vi "[ce] INI - RW Control Values.vi"(6 "cmd (load)":enum16{"load", "save"}(ring), 7 "Section":string="GENERAL", 8 "error in":errorcluster, 10 "Ctrl refnums":refnum<vi>[](array[refnum]), 11 "INI refnum":T1) -> (0 "error out":errorcluster, 3 "dup INI refnum":T1)   [LabVIEW 2021]
doc: "::: CalcExpress Toolkit :::\nCopyright (c) 2000-2026 Konstantin Shifershteyn. All rights reserved."
uses:
  <vilib>/Utility/config.llb/Config Data RefNum.ctl
  <vilib>/Utility/config.llb/Write Key (Path).vi
  <vilib>/Utility/config.llb/Write Key (String).vi
  <vilib>/Utility/config.llb/Write Key (Boolean).vi
  <vilib>/Utility/config.llb/Write Key (U32).vi
  <vilib>/Utility/config.llb/Write Key (I32).vi
  <vilib>/Utility/config.llb/Write Key (Double).vi
  <vilib>/Utility/config.llb/Read Key (Path).vi
  <vilib>/Utility/config.llb/Read Key (String).vi
  <vilib>/Utility/config.llb/Read Key (Boolean).vi
  <vilib>/Utility/config.llb/Read Key (U32).vi
  <vilib>/Utility/config.llb/Read Key (I32).vi
  <vilib>/Utility/config.llb/Read Key (Double).vi
  <vilib>/Utility/config.llb/NI_LVConfig.lvlib
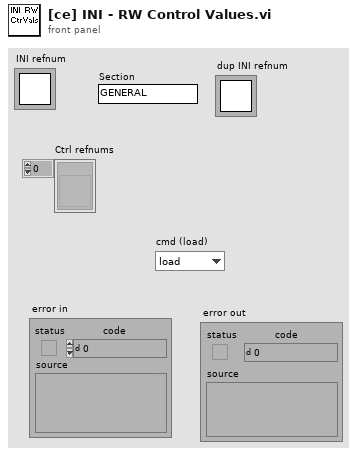
[diagram p1: front panel]
types:
  T1 = typedef "NI_LVConfig.lvlib/Config Data RefNum.ctl" = refnum<k1>
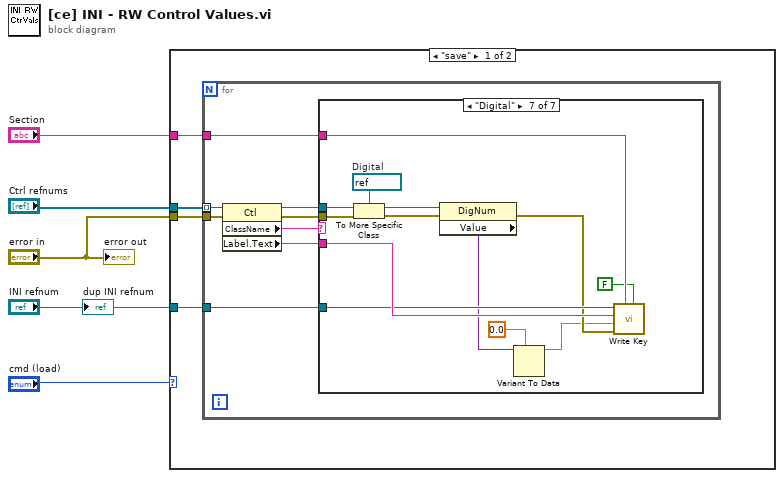
[diagram p0: block diagram]
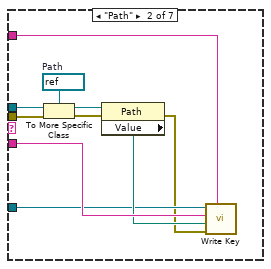
[diagram p3: hidden frame]
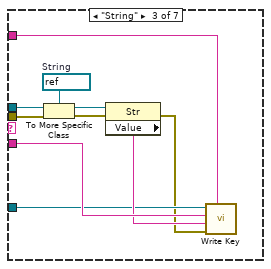
[diagram p4: hidden frame]
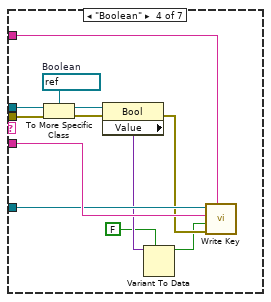
[diagram p5: hidden frame]
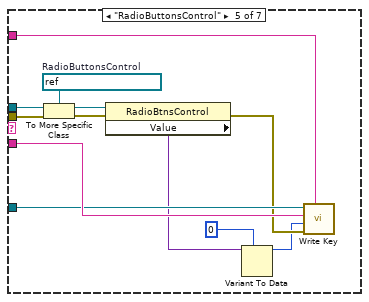
[diagram p6: hidden frame]
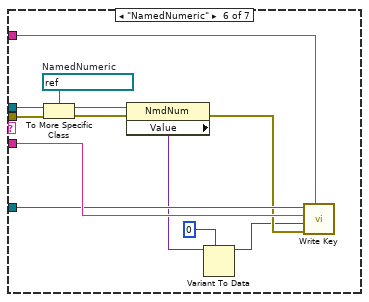
[diagram p7: hidden frame]
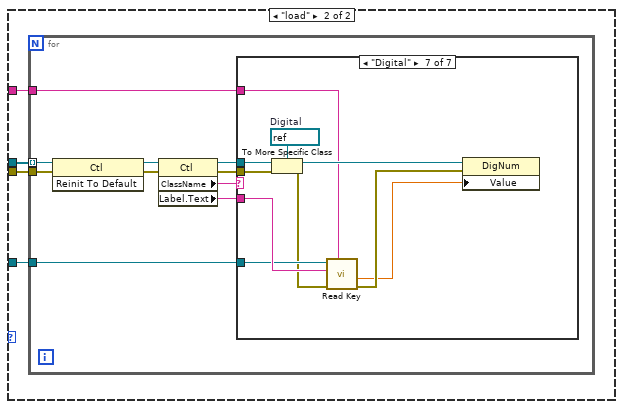
[diagram p8: hidden frame]
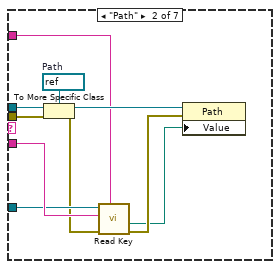
[diagram p10: hidden frame]
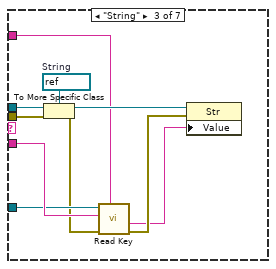
[diagram p11: hidden frame]
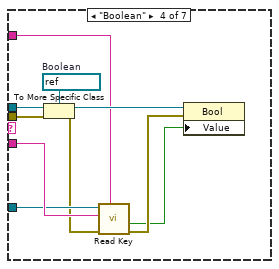
[diagram p12: hidden frame]
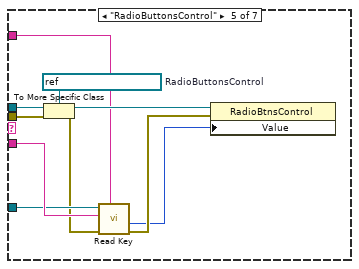
[diagram p13: hidden frame]
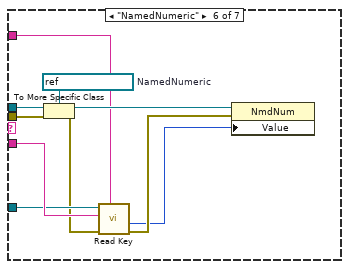
[diagram p14: hidden frame]
diagram:
  n1 = case shown="\"save\"" "cmd (load)" {
    tunnel: "Ctrl refnums" -> [w9 w92]
    tunnel: "error in" -> [w8 w91]
    tunnel: "INI refnum" -> [w7 w90]
    tunnel: "Section" -> [w6 w89]
    frame "save" {
      n2 = for {
        tunnel: w9 -> [w14] mode=indexing
        tunnel: w7 -> [w13]
        tunnel: w8 -> [w11]
        tunnel: w6 -> [w10]
        n3 = property class="Ctl"(reference=w14, error in=w11) -> (reference out=w16:refnum<vi>, error out=w12:errorcluster, "ClassName"=w17:string, "Label.Text"=w15:string)
        n4 = case shown="\"Digital\"" w17 {
          selector: w17 -> [w19 _ _ _ _ _ _]
          tunnel: w16 -> [_ w29 w39 w51 w63 w75 w88]
          tunnel: w15 -> [w18 w26 w36 w48 w60 w72 w85]
          tunnel: w13 -> [_ w24 w34 w47 w59 w71 w84]
          tunnel: w12 -> [_ w23 w33 w46 w58 w70 w83]
          tunnel: w10 -> [_ w20 w30 w43 w55 w67 w80]
          frame Default {
            n5 = flat-sequence {
              tunnel: w19 -> [_]
              tunnel: w18 -> [_]
              frame #0 {
              }
            }
          }
          frame "Path" {
            w27 = refnum<vi> refnum  # Path
            n6 = To More Specific Class(target class=w27, reference=w29, error in=w23) -> (specific class reference=w28:refnum<vi>, error out=w22:errorcluster)
            n7 = property class="Path"(reference=w28, error in=w22) -> (error out=w21:errorcluster, "Value"=w25:path)  [unwired: 1 out]
            n8 = call-poly <vilib>:"Write Key.vi"("section"=w20, "error in (no error)"=w21, "value"=w25, "key"=w26, "refnum"=w24) -> ()  [unwired: 4 in, 3 out]
          }
          frame "String" {
            w37 = refnum<vi> refnum  # String
            n9 = To More Specific Class(target class=w37, reference=w39, error in=w33) -> (specific class reference=w38:refnum<vi>, error out=w32:errorcluster)
            n10 = property class="Str"(reference=w38, error in=w32) -> (error out=w31:errorcluster, "Value"=w35:string)  [unwired: 1 out]
            n11 = call-poly <vilib>:"Write Key.vi"("section"=w30, "error in (no error)"=w31, "value"=w35, "key"=w36, "refnum"=w34) -> ()  [unwired: 4 in, 3 out]
          }
          frame "Boolean" {
            w49 = refnum<vi> refnum  # Boolean
            n12 = To More Specific Class(target class=w49, reference=w51, error in=w46) -> (specific class reference=w50:refnum<vi>, error out=w45:errorcluster)
            n13 = property class="Bool"(reference=w50, error in=w45) -> (error out=w44:errorcluster, "Value"=w42:variant)  [unwired: 1 out]
            n14 = Variant To Data(type=FALSE, Variant=w42) -> (data=w40:bool)  [unwired: 1 in, 1 out]
            n15 = call-poly <vilib>:"Write Key.vi"("section"=w43, "error in (no error)"=w44, "value"=w40, "key"=w48, "refnum"=w47) -> ()  [unwired: 4 in, 3 out]
          }
          frame "RadioButtonsControl" {
            w61 = refnum<vi> refnum  # RadioButtonsControl
            n16 = To More Specific Class(target class=w61, reference=w63, error in=w58) -> (specific class reference=w62:refnum<vi>, error out=w57:errorcluster)
            n17 = property class="RadioBtnsControl"(reference=w62, error in=w57) -> (error out=w56:errorcluster, "Value"=w54:variant)  [unwired: 1 out]
            n18 = Variant To Data(type=u32 0, Variant=w54) -> (data=w52:u32)  [unwired: 1 in, 1 out]
            n19 = call-poly <vilib>:"Write Key.vi"("section"=w55, "error in (no error)"=w56, "value"=w52, "key"=w60, "refnum"=w59) -> ()  [unwired: 4 in, 3 out]
          }
          frame "NamedNumeric" {
            w73 = refnum<vi> refnum  # NamedNumeric
            n20 = To More Specific Class(target class=w73, reference=w75, error in=w70) -> (specific class reference=w74:refnum<vi>, error out=w69:errorcluster)
            n21 = property class="NmdNum"(reference=w74, error in=w69) -> (error out=w68:errorcluster, "Value"=w66:variant)  [unwired: 1 out]
            n22 = Variant To Data(type=0, Variant=w66) -> (data=w64:i32)  [unwired: 1 in, 1 out]
            n23 = call-poly <vilib>:"Write Key.vi"("section"=w67, "error in (no error)"=w68, "value"=w64, "key"=w72, "refnum"=w71) -> ()  [unwired: 4 in, 3 out]
          }
          frame "Digital" {
            w86 = refnum<vi> refnum  # Digital
            n24 = To More Specific Class(target class=w86, reference=w88, error in=w83) -> (specific class reference=w87:refnum<vi>, error out=w82:errorcluster)
            n25 = property class="DigNum"(reference=w87, error in=w82) -> (error out=w81:errorcluster, "Value"=w79:variant)  [unwired: 1 out]
            n26 = Variant To Data(type=0.0, Variant=w79) -> (data=w77:dbl)  [unwired: 1 in, 1 out]
            n27 = call-poly <vilib>:"Write Key.vi"("use system decimal point (T)"=FALSE, "section"=w80, "error in (no error)"=w81, "value"=w77, "key"=w85, "refnum"=w84) -> ()  [unwired: 3 in, 3 out]
          }
        }
      }
    }
    frame "load" {
      n28 = for {
        tunnel: w92 -> [w96] mode=indexing
        tunnel: w90 -> [w99]
        tunnel: w91 -> [w94]
        tunnel: w89 -> [w97]
        n29 = invoke class="Ctl" method="Reinit To Default"(reference=w96, error in=w94) -> (reference out=w95:refnum<vi>, error out=w93:errorcluster)  [unwired: 1 in, 1 out]
        n30 = property class="Ctl"(reference=w95, error in=w93) -> (reference out=w101:refnum<vi>, error out=w98:errorcluster, "ClassName"=w102:string, "Label.Text"=w100:string)
        n31 = case shown="\"Digital\"" w102 {
          tunnel: w101 -> [_ w112 w122 w132 w142 w152 w162]
          tunnel: w100 -> [_ w109 w119 w129 w139 w149 w159]
          tunnel: w99 -> [_ w108 w118 w128 w138 w148 w158]
          tunnel: w98 -> [_ w107 w117 w127 w137 w147 w157]
          tunnel: w97 -> [_ w104 w114 w124 w134 w144 w154]
          frame Default {
          }
          frame "Path" {
            w110 = refnum<vi> refnum  # Path
            n32 = To More Specific Class(target class=w110, reference=w112, error in=w107) -> (specific class reference=w111:refnum<vi>, error out=w106:errorcluster)
            n33 = call-poly <vilib>:"Read Key.vi"("section"=w104, "error in (no error)"=w106, "key"=w109, "refnum"=w108) -> ("error out"=w105:errorcluster, "value"=w103:path)  [unwired: 4 in, 2 out]
            n34 = property class="Path"(reference=w111, error in=w105, "Value"=w103) -> ()  [unwired: 2 out]
          }
          frame "String" {
            w120 = refnum<vi> refnum  # String
            n35 = To More Specific Class(target class=w120, reference=w122, error in=w117) -> (specific class reference=w121:refnum<vi>, error out=w116:errorcluster)
            n36 = call-poly <vilib>:"Read Key.vi"("section"=w114, "error in (no error)"=w116, "key"=w119, "refnum"=w118) -> ("error out"=w115:errorcluster, "value"=w113:string)  [unwired: 4 in, 2 out]
            n37 = property class="Str"(reference=w121, error in=w115, "Value"=w113) -> ()  [unwired: 2 out]
          }
          frame "Boolean" {
            w130 = refnum<vi> refnum  # Boolean
            n38 = To More Specific Class(target class=w130, reference=w132, error in=w127) -> (specific class reference=w131:refnum<vi>, error out=w126:errorcluster)
            n39 = call-poly <vilib>:"Read Key.vi"("section"=w124, "error in (no error)"=w126, "key"=w129, "refnum"=w128) -> ("error out"=w125:errorcluster, "value"=w123:bool)  [unwired: 4 in, 2 out]
            n40 = property class="Bool"(reference=w131, error in=w125, "Value"=w123) -> ()  [unwired: 2 out]
          }
          frame "RadioButtonsControl" {
            w140 = refnum<vi> refnum  # RadioButtonsControl
            n41 = To More Specific Class(target class=w140, reference=w142, error in=w137) -> (specific class reference=w141:refnum<vi>, error out=w136:errorcluster)
            n42 = call-poly <vilib>:"Read Key.vi"("section"=w134, "error in (no error)"=w136, "key"=w139, "refnum"=w138) -> ("error out"=w135:errorcluster, "value"=w133:u32)  [unwired: 4 in, 2 out]
            n43 = property class="RadioBtnsControl"(reference=w141, error in=w135, "Value"=w133) -> ()  [unwired: 2 out]
          }
          frame "NamedNumeric" {
            w150 = refnum<vi> refnum  # NamedNumeric
            n44 = To More Specific Class(target class=w150, reference=w152, error in=w147) -> (specific class reference=w151:refnum<vi>, error out=w146:errorcluster)
            n45 = call-poly <vilib>:"Read Key.vi"("section"=w144, "error in (no error)"=w146, "key"=w149, "refnum"=w148) -> ("error out"=w145:errorcluster, "value"=w143:i32)  [unwired: 4 in, 2 out]
            n46 = property class="NmdNum"(reference=w151, error in=w145, "Value"=w143) -> ()  [unwired: 2 out]
          }
          frame "Digital" {
            w160 = refnum<vi> refnum  # Digital
            n47 = To More Specific Class(target class=w160, reference=w162, error in=w157) -> (specific class reference=w161:refnum<vi>, error out=w156:errorcluster)
            n48 = call-poly <vilib>:"Read Key.vi"("section"=w154, "error in (no error)"=w156, "key"=w159, "refnum"=w158) -> ("error out"=w155:errorcluster, "value"=w153:dbl)  [unwired: 4 in, 2 out]
            n49 = property class="DigNum"(reference=w161, error in=w155, "Value"=w153) -> ()  [unwired: 2 out]
          }
        }
      }
    }
  }
  "error out" <- "error in"
  "dup INI refnum" <- "INI refnum"
